vi "IDS Preview Capture.vi"(8 "Image Ref":T1, 9 "IDS Camera Ref":refnum<k24>, 10 "IDS Actions":T2, 11 "IDS Notifier":refnum<notifier>) -> (0 "Error":errorcluster, 3 "IDS Notifier":refnum<notifier>)   [LabVIEW 2016]
uses:
  IDS Controls/IDS Actions.ctl
  IDS Controls/IDS Notifier Element.ctl
  IDS Controls/IDS Parameters.ctl
  IDS Controls/IDS Parameter List.ctl
  IDS Controls/IDS ROI.ctl
  <vilib>/vision/Image Controls.llb/IMAQ Image.ctl
  C:/Users/Ries Lab/Documents/Microscope Control from Sheng Account/Microscope-Control/Device Library/Cameras/IDS/IDS LabView Examples/LabVIEW/ueye.NET/uEyeDotNet.dll
  IDS LabView Examples/LabVIEW/ueye.NET/uEyeDotNet.dll
  Tools/TIFF Image Read and Write/ImageJ TIF Type Defs/TIF Write Image Information.ctl
  Camera Controls/Camera IMAQ Key Info.ctl
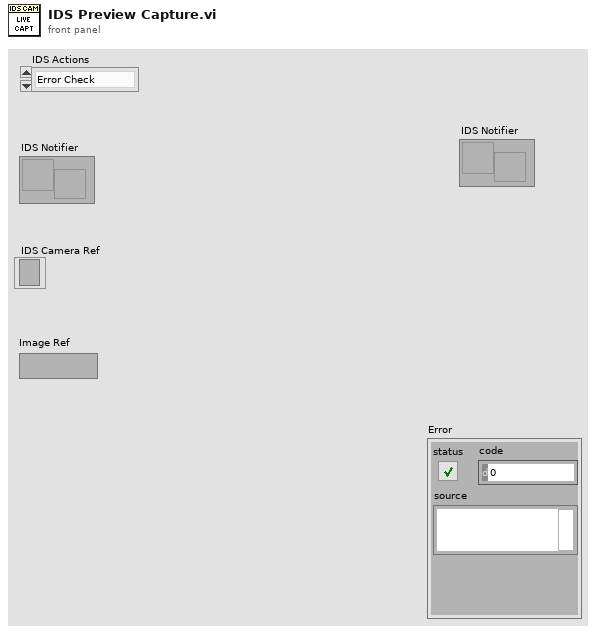
[diagram p1: front panel]
types:
  T1 = typedef "IMAQ Image.ctl" = refnum<image>
  T2 = typedef "IDS Actions.ctl" = enum16{"Error Check", "Initialize", "Preview", "Record", "Abort", "Record Settings", "Set Parameter", "Get Parameter", "Set ROI", "Get ROI", "Status", "Quit"}
  T3 = typedef "Camera IMAQ Key Info.ctl" = cluster{"Frame":u32, "Sensor Height":i32, "Sensor Width":i32, "ROI Height":i32, "ROI Width":i32, "ROI Enable?":bool, "Bit per Pixel":u8}
  T4 = typedef "TIF Write Image Information.ctl" = cluster{"Image Width (Pixels)":u32, "Image Height (Pixels)":u32, "Pixel Width (µm)":dbl, "Pixel Height (µm)":dbl, "Bits Per Sample (e.g. 16)":u32, "No. of Frames":u32, "No. of Slices":u32, "Time Step (sec)":dbl, "Z Step (µm)":dbl}
  T5 = typedef "IDS Notifier Element.ctl" = cluster{"IDS Actions":T2, "Received?":bool, "IDS Parameter":T6, "IDS ROI":T8, "Running?":bool, "File Path":path, "# of frames":u32, "Image Ref":T1, "Error":errorcluster}
  T6 = typedef "IDS Parameters.ctl" = cluster{"Parameter":T7, "Value":dbl}
  T7 = typedef "IDS Parameter List.ctl" = enum16{"Exposure Time (s)"}
  T8 = typedef "IDS ROI.ctl" = cluster{"H Offset":i32, "V Offset":i32, "H Width":i32, "V Width":i32}
  T9 = enum16{"big-endian, network order", "native, host order", "little-endian"}
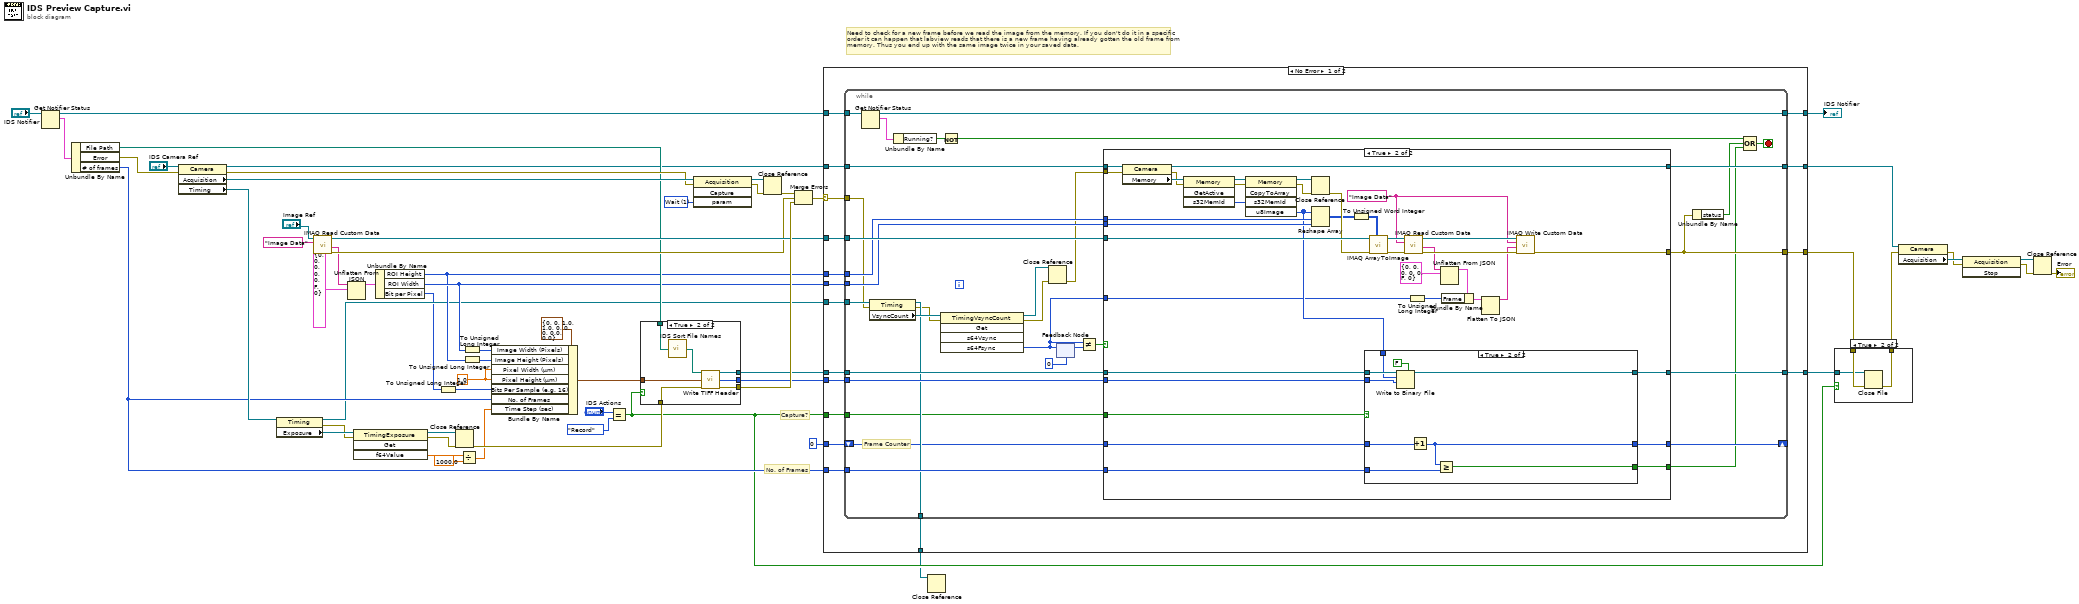
[diagram p0: block diagram]
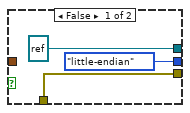
[diagram p3: hidden frame]
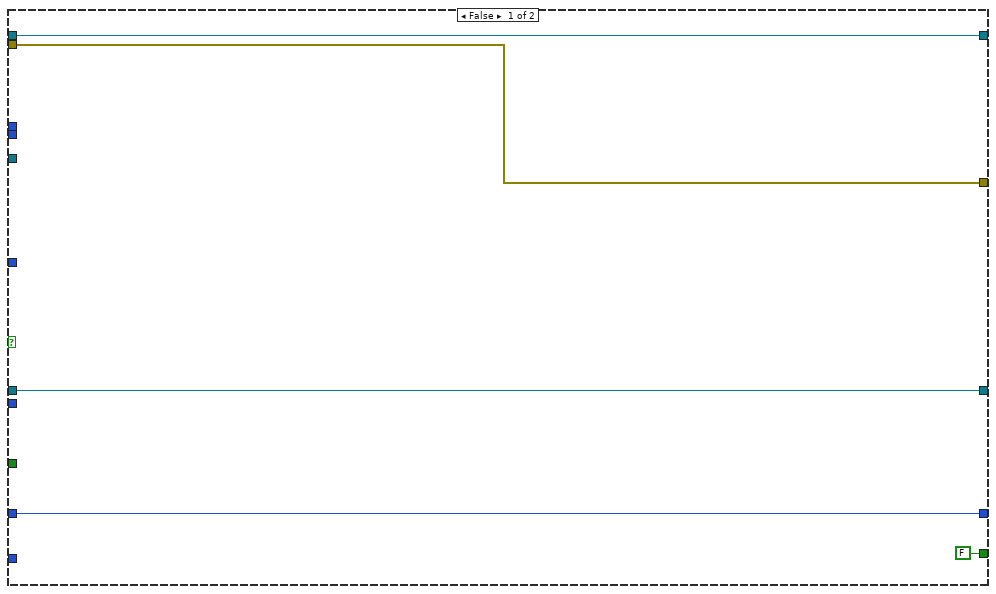
[diagram p4: hidden frame]
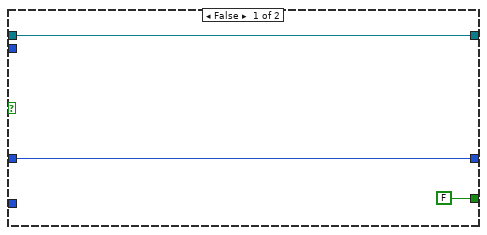
[diagram p5: hidden frame]
diagram:
  w8 = 1 items=["DontWait"=0, "Wait"=1, "Force"=16384] ("param")
  w34 = 1.0 ("Pixel Height (µm)")
  # "Need to check for a new frame before we read the image from the memory. If you don't do it in a specific\norder it can happen that labview reads that there is a new frame having already gotten the old frame from\nmemory. Thus you end up with the same image twice in your saved data."
  # "Capture?"
  # "No. of Frames"
  n1 = Get Notifier Status(notifier="IDS Notifier") -> (notifier out=w42:refnum<notifier>, current notification=w41:T5)  [unwired: 1 in, 3 out]
  n2 = Unbundle By Name(w41) -> ("File Path"=w18:path, "Error"=w29:errorcluster, "# of frames"=w19:u32)
  n3 = property class="Camera"(reference="IDS Camera Ref", error in=w29) -> (reference out=w7:refnum<k24>, error out=w58:errorcluster, "Acquisition"=w59:refnum<k24>, "Timing"=w28:refnum<k24>)
  n4 = property class="Timing"(reference=w28) -> (reference out=w10:refnum<k24>, error out=w11:errorcluster, "Exposure"=w27:refnum<k24>)  [unwired: 1 in]
  n5 = call "IMAQ Read Custom Data"("Key"="Image Data", "Image"="Image Ref") -> ("error out"=w25:errorcluster, "Custom Data Out"=w23:string, "Image (duplicate)"=w26:T1)  [unwired: 7 in]
  n6 = Unflatten From JSON(JSON string=w23, type and defaults=T3 {"Frame"=0, "Sensor Height"=0, "Sensor Width"=0, "ROI Height"=0, "ROI Width"=0, "ROI Enable?"=FALSE, "Bit per Pixel"=0} ("Camera IMAQ Key Info")) -> (value=w22:T3)  [unwired: 5 in, 1 out]
  n7 = invoke class="TimingExposure" method="Get"(reference=w27, error in=w11) -> (reference out=w32:refnum<k24>, error out=w31:errorcluster, "f64Value"=w4:dbl)  [unwired: 2 in, 1 out]
  n8 = Unbundle By Name(w22) -> ("ROI Height"=w16:i32, "ROI Width"=w17:i32, "Bit per Pixel"=w6:u8)
  n9 = To Unsigned Long Integer(number=w6) -> (unsigned 32bit integer=w1:u32)
  n10 = Close Reference(reference=w32, error in (no error)=w31) -> (error out=w30:errorcluster)
  n11 = Divide(x=w4, y=1000.0) -> (x/y=w2:dbl)
  n12 = To Unsigned Long Integer(number=w17) -> (unsigned 32bit integer=w36:u32)
  n13 = To Unsigned Long Integer(number=w16) -> (unsigned 32bit integer=w35:u32)
  n14 = Bundle By Name(cluster=T4 {"Image Width (Pixels)"=0, "Image Height (Pixels)"=0, "Pixel Width (µm)"=1.0, "Pixel Height (µm)"=1.0, "Bits Per Sample (e.g. 16)"=0, "No. of Frames"=0, "No. of Slices"=0, "Time Step (sec)"=0.0, "Z Step (µm)"=0.0} ("Image Info"), "Image Width (Pixels)"=w36, "Image Height (Pixels)"=w35, "Pixel Width (µm)"=w34, "Pixel Height (µm)"=w34, "Bits Per Sample (e.g. 16)"=w1, "No. of Frames"=w19, "Time Step (sec)"=w2) -> (w37:T4)
  n15 = Equal?(x="IDS Actions", y=IDS_Actions."Record") -> (x = y?=w12:bool)
  n16 = case shown="True" w12 {
    tunnel: w37 -> [_ w69]
    tunnel: w18 -> [_ w64]
    tunnel: [w62 w68] -> w33
    tunnel: w30 -> [w62 w67]
    tunnel: [refnum<file> refnum ("File Ref") w66] -> w20
    tunnel: [T9."little-endian" ("Byte Order") w65] -> w21
    frame False {
    }
    frame True {
      n17 = call "IDS Sort File Names.vi"("Requested File Path"=w64) -> ("Resulting File Path"=w63:path)  [unwired: 14 in]
      n18 = call "Write TIFF Header.vi"("File Path"=w63, "Image Info"=w69, "Error"=w67) -> ("File Ref"=w66:refnum<file>, "Byte Order"=w65:T9, "Error"=w68:errorcluster)  [unwired: 10 in]
    }
  }
  n19 = invoke class="Acquisition" method="Capture"(reference=w59, error in=w58, "param"=w8) -> (reference out=w57:refnum<k24>, error out=w56:errorcluster)  [unwired: 1 in, 2 out]
  n20 = Close Reference(reference=w57, error in (no error)=w56) -> (error out=w55:errorcluster)
  n21 = Merge Errors(w55, w25, w33) -> (w54:errorcluster)
  n22 = case shown="No Error" w54 {
    selector: w54 -> [w82 w179]
    tunnel: w42 -> [w86 w177]
    tunnel: [w80 w177] -> w45
    tunnel: w7 -> [w85 w178]
    tunnel: w16 -> [w84 _]
    tunnel: w17 -> [w83 _]
    tunnel: w26 -> [w81 _]
    tunnel: [w79 w179] -> w14
    tunnel: [w78 w178] -> w52
    tunnel: w12 -> [w77 _]
    tunnel: w21 -> [w76 _]
    tunnel: w20 -> [w75 w176]
    tunnel: w19 -> [w74 _]
    tunnel: [w73 w176] -> w15
    tunnel: w10 -> [w72 w175]
    tunnel: [w71 w175] -> w9
    tunnel: u32 0 ("s64Fsync") -> [w70 _]
    frame No Error {
      n23 = while {
        tunnel: w86 -> [w119]
        tunnel: w85 -> [w118]
        tunnel: w84 -> [w115]
        tunnel: w83 -> [w114]
        tunnel: w82 -> [w96]
        tunnel: [w117] -> w78
        tunnel: w81 -> [w116]
        tunnel: [w113] -> w80
        tunnel: [w111] -> w79
        tunnel: w77 -> [w91]
        tunnel: w76 -> [w107]
        tunnel: w75 -> [w108]
        tunnel: w74 -> [w109]
        tunnel: [w103] -> w73
        tunnel: w72 -> [w101]
        tunnel: [w98] -> w71
        shift-right: [w94] -> _
        shift-left: w70 -> [w95]
        stop <- w104 stop-if-true
        # "Frame Counter"
        n24 = Get Notifier Status(notifier=w119) -> (notifier out=w113:refnum<notifier>, current notification=w110:T5)  [unwired: 1 in, 3 out]
        n25 = property class="Timing"(reference=w101, error in=w96) -> (reference out=w98:refnum<k24>, error out=w92:errorcluster, "VsyncCount"=w102:refnum<k24>)
        n26 = Unbundle By Name(w110) -> ("Running?"=w112:bool)
        n27 = invoke class="TimingVsyncCount" method="Get"(reference=w102, error in=w92) -> (reference out=w87:refnum<k24>, error out=w89:errorcluster, "s64Fsync"=w97:i64)  [unwired: 3 in, 2 out]
        n28 = Not(x=w112) -> (.not. x?=w106:bool)
        n29 = Close Reference(reference=w87, error in (no error)=w89) -> (error out=w88:errorcluster)
        n30 = feedback #1(i64 0 ("s64Fsync")) -> (w99:i64)
        n31 = feedback-in #1(w97) -> ()
        n32 = Not Equal?(x=w97, y=w99) -> (x != y?=w90:bool)
        n33 = case shown="True" w90 {
          tunnel: w118 -> [w124 w162]
          tunnel: [w124 w154] -> w117
          tunnel: w116 -> [_ w153]
          tunnel: w115 -> [_ w152]
          tunnel: w114 -> [_ w151]
          tunnel: [w123 w149] -> w111
          tunnel: w109 -> [_ w138]
          tunnel: w108 -> [w120 w137]
          tunnel: w107 -> [_ w136]
          tunnel: [w120 w132] -> w103
          tunnel: w97 -> [_ w130]
          tunnel: w88 -> [w123 w129]
          tunnel: w95 -> [w122 w128]
          tunnel: [w122 w127] -> w94
          tunnel: [FALSE w126] -> w93
          tunnel: w91 -> [_ w125]
          frame False {
          }
          frame True {
            w144 = "Image Data" ("Key")
            n34 = property class="Camera"(reference=w162, error in=w129) -> (reference out=w154:refnum<k24>, error out=w160:errorcluster, "Memory"=w161:refnum<k24>)
            n35 = invoke class="Memory" method="GetActive"(reference=w161, error in=w160) -> (reference out=w159:refnum<k24>, error out=w157:errorcluster, "s32MemId"=w158:i32)  [unwired: 2 in, 1 out]
            n36 = invoke class="Memory" method="CopyToArray"(reference=w159, error in=w157, "s32MemId"=w158) -> (reference out=w156:refnum<k24>, error out=w155:errorcluster, "u8Image"=w133:u8[])  [unwired: 2 in, 2 out]
            n37 = Close Reference(reference=w156, error in (no error)=w155) -> (error out=w150:errorcluster)
            n38 = Reshape Array(w133, w152, w151) -> (w134:u8[][])
            n39 = To Unsigned Word Integer(number=w134) -> (unsigned 16bit integer=w135:u16[][])
            n40 = case shown="True" w125 {
              tunnel: w138 -> [_ w174]
              tunnel: w137 -> [w165 w170]
              tunnel: w136 -> [_ w173]
              tunnel: [w165 w171] -> w132
              tunnel: w133 -> [_ w169]
              tunnel: w128 -> [w164 w168]
              tunnel: [w164 w167] -> w127
              tunnel: [FALSE w166] -> w126
              frame False {
              }
              frame True {
                n41 = Write to Binary File(file (use dialog)=w170, data=w169, 5:FALSE ("prepend array or string size? (T)"), 9:w173) -> (refnum out=w171:refnum<file>)  [unwired: 2 in, 2 out]
                n42 = Increment(x=w168) -> (x+1=w167:u32)
                n43 = Greater Or Equal?(x=w167, y=w174) -> (x >= y?=w166:bool)
              }
            }
            n44 = call "IMAQ ArrayToImage"("Image Pixels (U16)"=w135, "error in (no error)"=w150, "Image"=w153) -> ("error out"=w146:errorcluster, "Image Out"=w148:T1)  [unwired: 7 in]
            n45 = call "IMAQ Read Custom Data"("error in (no error)"=w146, "Key"=w144, "Image"=w148) -> ("error out"=w145:errorcluster, "Custom Data Out"=w143:string, "Image (duplicate)"=w147:T1)  [unwired: 6 in]
            n46 = To Unsigned Long Integer(number=w130) -> (unsigned 32bit integer=w131:u32)
            n47 = Unflatten From JSON(JSON string=w143, type and defaults=T3 {"Frame"=0, "Sensor Height"=0, "Sensor Width"=0, "ROI Height"=0, "ROI Width"=0, "ROI Enable?"=FALSE, "Bit per Pixel"=0} ("Camera IMAQ Key Info")) -> (value=w141:T3)  [unwired: 5 in, 1 out]
            n48 = Bundle By Name(cluster=w141, "Frame"=w131) -> (w140:T3)
            n49 = Flatten To JSON(anything=w140) -> (JSON string=w139:string)  [unwired: 2 in, 1 out]
            n50 = call "IMAQ Write Custom Data"("error in (no error)"=w145, "Custom Data In"=w139, "Key"=w144, "Image"=w147) -> ("error out"=w149:errorcluster)  [unwired: 6 in, 1 out]
          }
        }
        n51 = Unbundle By Name(w111) -> ("status"=w105:bool)
        n52 = Compound Arithmetic op=OR(w106, w105, w93) -> (w104:bool)
      }
    }
    frame Error {
    }
  }
  "IDS Notifier" <- w45
  n53 = Close Reference(reference=w9) -> ()  [unwired: 1 in, 1 out]
  n54 = case shown="True" w12 {
    tunnel: w15 -> [_ w181]
    tunnel: w14 -> [w180 w183]
    tunnel: [w180 w182] -> w13
    frame False {
    }
    frame True {
      n55 = Close File(refnum=w181, error in=w183) -> (error out=w182:errorcluster)  [unwired: 1 out]
    }
  }
  n56 = property class="Camera"(reference=w52, error in=w13) -> (error out=w50:errorcluster, "Acquisition"=w51:refnum<k24>)  [unwired: 1 out]
  n57 = invoke class="Acquisition" method="Stop"(reference=w51, error in=w50) -> (reference out=w49:refnum<k24>, error out=w48:errorcluster)  [unwired: 1 in, 1 out]
  n58 = Close Reference(reference=w49, error in (no error)=w48) -> (error out=→"Error":errorcluster)
